vi "Wait Until Cancelled or Complete.vi"(6 "done channel":T1, 8 "error in (no error)":errorcluster, 9 "ms polling interval":i32=100, 10 "scope session":refnum<k15>, 11 "measure call context in":refnum<class "Measure Call Context.lvclass">) -> (0 "error out":errorcluster, 3 "measure call context out":refnum<class "Measure Call Context.lvclass">)   [LabVIEW 2021, in "NIScopeAcquireWaveform.lvlib"]
doc: "Monitor for cancellation and abort the acquisition if a request to cancel the measurement is received before a trigger."
uses:
  NIScopeAcquireWaveform.lvlib
  <vilib>/Plug-In SDKs/Measurements/Measure Call Context/Measure Call Context.lvclass
  <extravilib>/ChannelInstances/Event Messenger-bool/))Channel.ctl
  <extravilib>/ChannelInstances/Event Messenger-bool/))Channel.vi
  <extravilib>/ChannelInstances/Event Messenger-bool.lvlib
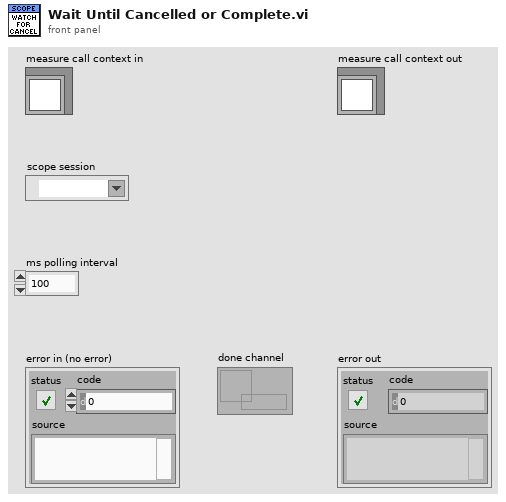
[diagram p1: front panel]
types:
  T1 = typedef "Event Messenger-bool.lvlib/))Channel.ctl" = refnum<queue>
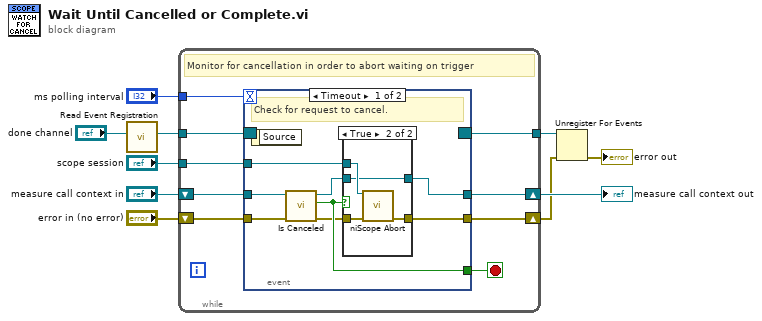
[diagram p0: block diagram]
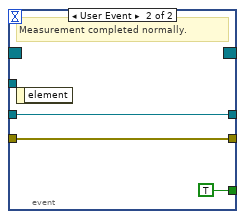
[diagram p3: hidden frame]
diagram:
  n1 = call <extravilib>:"Read Event Registration.vi"("channel"="done channel") -> ("event registration refnum"=w4:refnum<event-registration>)  [unwired: 10 in]
  n2 = while {
    tunnel: "scope session" -> [w17]
    shift-right: [w18] -> w9
    shift-left: "measure call context in" -> [w19]
    tunnel: "ms polling interval" -> [w13]
    shift-right: [w14] -> w2
    shift-left: "error in (no error)" -> [w15]
    tunnel: w4 -> [w12]
    tunnel: [w11] -> w3
    stop <- w16 stop-if-true
    # "Monitor for cancellation in order to abort waiting on trigger"
    n3 = event shown="[0] Timeout" {
      selector: w12 -> [_ _]
      dyn-events: [_ _] -> w11
      timeout: w13 -> [_ _]
      tunnel: w19 -> [w27 w34]
      tunnel: [w26 w34] -> w18
      tunnel: w17 -> [w25 _]
      tunnel: [w24 TRUE ("is canceled?")] -> w16
      tunnel: w15 -> [w23 w35]
      tunnel: [w22 w35] -> w14
      event Timeout {
        # "Check for request to cancel."
        n4 = event-data() -> ()  [unwired: 1 in, 1 out]
        n5 = call <vilib>:"Is Canceled.vi"("error in"=w23, "measure call context in"=w27) -> ("error out"=w21:errorcluster, "is canceled?"=w24:bool, "measure call context out"=w20:refnum<class "Measure Call Context.lvclass">)  [unwired: 7 in]
        n6 = case shown="True" w24 {
          tunnel: w21 -> [w29 w33]
          tunnel: w20 -> [w28 w30]
          tunnel: [w29 w32] -> w22
          tunnel: [w28 w30] -> w26
          tunnel: w25 -> [_ w31]
          frame False {
          }
          frame True {
            n7 = call <instrlib>:"niScope Abort.vi"("instrument handle"=w31, "error in"=w33) -> ("error out"=w32:errorcluster)  [unwired: 12 in, 1 out]
          }
        }
      }
      event User Event {
        # "Measurement completed normally."
        n8 = event-data() -> ()  [unwired: 1 in, 1 out]
      }
    }
  }
  "measure call context out" <- w9
  n9 = Unregister For Events(event registration refnum=w3, error in=w2) -> (error out=→"error out":errorcluster)
